vi "Routing Channel Page.vi"(8 "error in (no error)":errorcluster, 11 "Node Ptr":T6 format="%.0x") -> (0 "error out":errorcluster)   [LabVIEW 2020, in "Routing and Faulting System Explorer.lvlib"]
uses:
  Routing and Faulting System Explorer.lvlib
  <vilib>/NI VeriStand/Custom Device API/Custom Device API.lvlib
  Scripting/Routing and Faulting Scripting.lvlib
  Routing Channel Page Controls.ctl
  Shared/UI Common/UI Common.lvlib
  2402a215-ce2b-4427-ab28-3f6d8102afb6.vi
  Shared/Constants.vi
  Shared/Routing and Faulting Shared.lvlib
  <vilib>/NI VeriStand/Custom Device API/Custom Device Item Ref.ctl
  State Control.ctl
  State-Value Row.ctl
  Connection Row.ctl
  Shared/UI Common/Add Button.ctl
panel:
  in  "Configuration Tab":T1(tab)
  in  "Connections":T2[](array[typedef])
  in  "State Value":string
  in  "State Description":string
  in  "Add Connection":T3
  in  "State Name":T4
  in  "Duplicate State":bool
  in  "Remove State":bool
  in  "Add State":bool
  in  "Previous State":bool
  in  "Next State":bool
  in  "States":T5[](array[typedef])
  in  "Initial State":string(combo)
  in  "Routing Channel Name":string
  in  "SHDocVw.IWebBrowser":refnum<k7>(container)
  in  "Description":string
  # "Source"
  # "Destination"
  # "State Name"
  # "State Value"
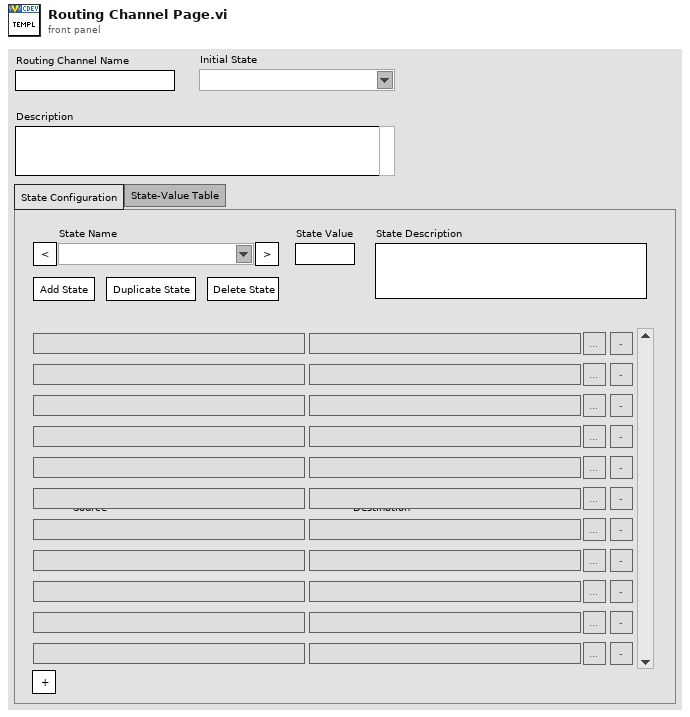
[diagram p1: front panel]
types:
  T1 = enum32{"State Configuration", "State-Value Table"}
  T2 = typedef "Routing and Faulting System Explorer.lvlib/Connection Row.ctl" = cluster{"Source":string, "Destination":string, "Edit":bool, "Remove":bool}
  T3 = typedef "UI Common.lvlib/Add Button.ctl" = bool
  T4 = typedef "Routing and Faulting System Explorer.lvlib/State Control.ctl" = string
  T5 = typedef "Routing and Faulting System Explorer.lvlib/State-Value Row.ctl" = cluster{"State":string, "State Value":string}
  T6 = typedef "Custom Device API.lvlib/Custom Device Item Ref.ctl" = u64
  T7 = typedef "Routing and Faulting System Explorer.lvlib/Routing Channel Page Controls.ctl" = cluster{"Description":refnum<vi>, "Routing Channel Name":refnum<vi>, "Initial State":refnum<vi>, "Configuration Tab":refnum<vi>, "States":refnum<vi>, "State Value":refnum<vi>, "State Name":refnum<vi>, "State Description":refnum<vi>, "Connections":refnum<vi>}
  T8 = typedef "Routing and Faulting Scripting.lvlib/Module Information.ctl" = cluster{"Module Path":string, "Product Name":string, "Possible Connections":T9[], "Configuration Revision":u32, "Validated":bool, "Missing":bool}
  T9 = typedef "Routing and Faulting Hardware API.lvlib/Possible Connections for Endpoint.ctl" = cluster{"Source":string, "Destinations":string[]}
  T10 = typedef "Routing and Faulting System Explorer.lvlib/Channel Editor State.ctl" = cluster{"Modules and Connections":T11[], "Alias Mappings UI":T12[], "Mappings by Module UI":T14[]}
  T11 = typedef "Routing and Faulting System Explorer.lvlib/Possible Connections.ctl" = cluster{" Module Path":string, "Short Module Path":string, "Product Name":string, "Possible Connections":T9[], "Missing":bool}
  T12 = typedef "Routing and Faulting Shared.lvlib/Alias Mapping.ctl" = cluster{"Alias":string, "Endpoint":T13}
  T13 = typedef "Routing and Faulting Shared.lvlib/Alias Endpoint.ctl" = cluster{"Module Path":string, "Endpoint":string}
  T14 = typedef "Routing and Faulting System Explorer.lvlib/Alias Map by Module.ctl" = cluster{"Module":string, "Alias Map":cluster{"Aliases":string[], "Endpoints":string[]}}
  T15 = typedef "Custom Device API.lvlib/Custom Device Commands.ctl" = enum16{"Default", "Item renamed", "Shutdown", "Dynamic button pressed"}
  T16 = typedef "Routing and Faulting Shared.lvlib/Connection.ctl" = cluster{"Module":string, "Source":string, "Destination":string}
  T17 = typedef "LVPoint32TypeDef.ctl" = cluster{"Horizontal":i32, "Vertical":i32}
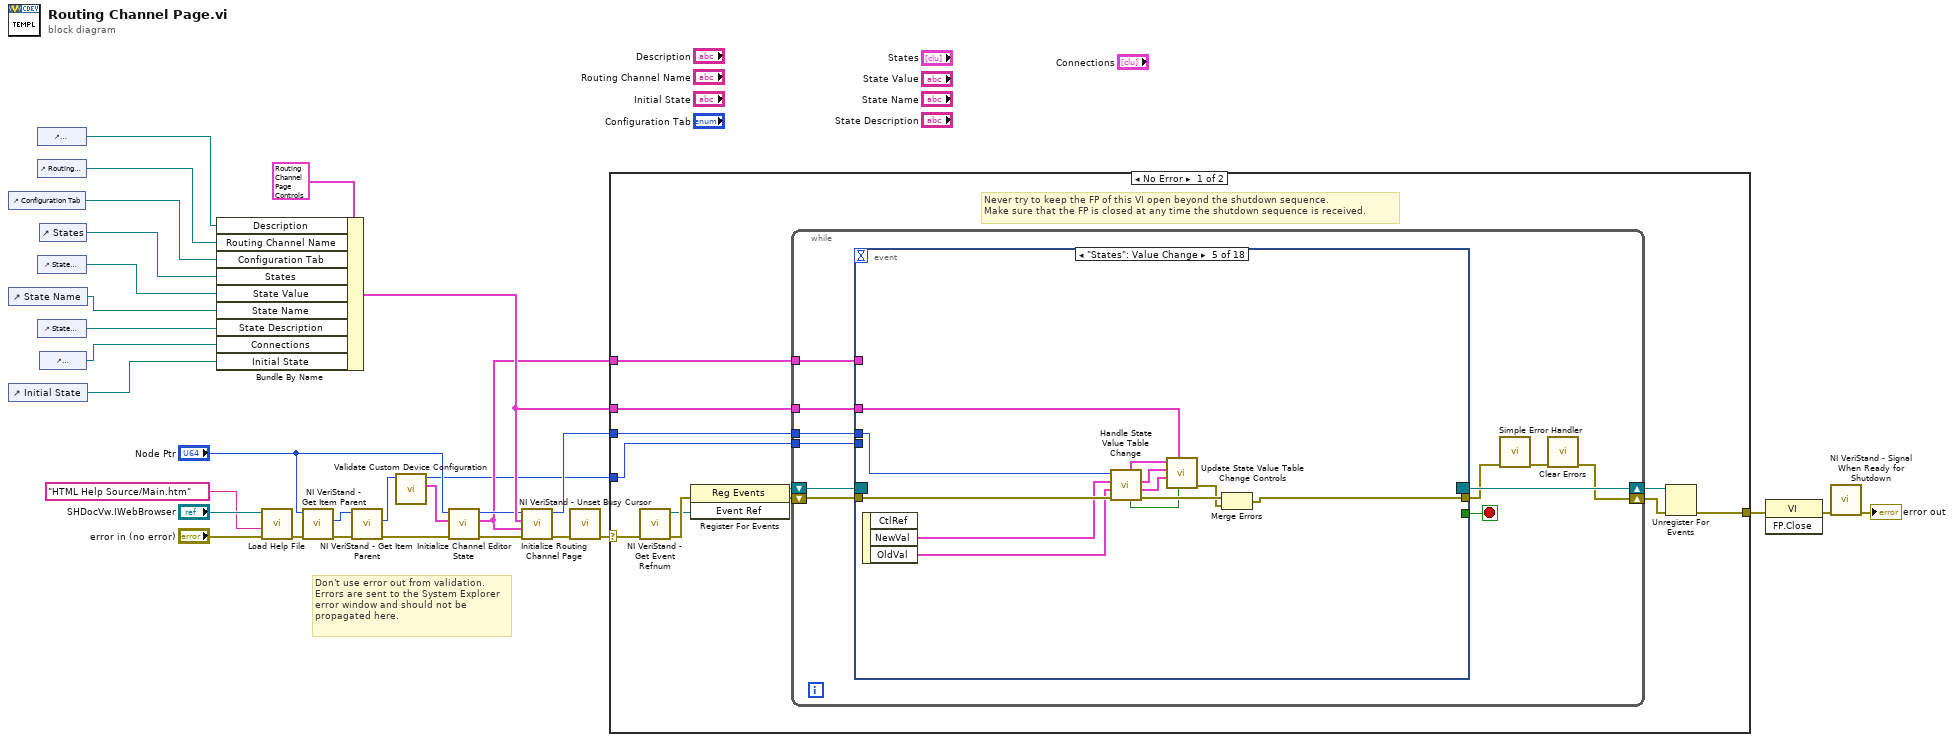
[diagram p0: block diagram]
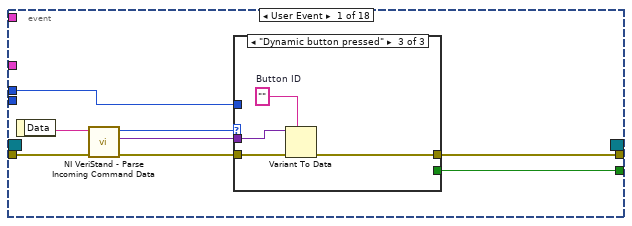
[diagram p2: hidden frame]
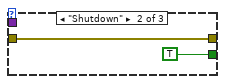
[diagram p4: hidden frame]
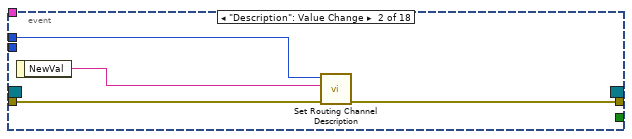
[diagram p5: hidden frame]
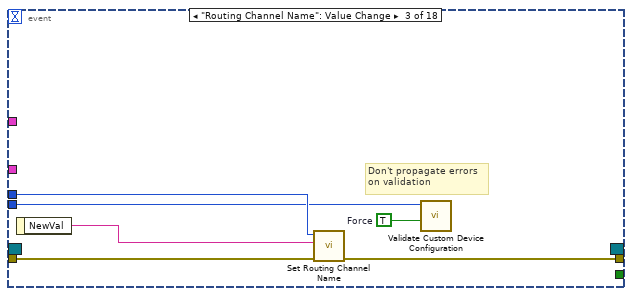
[diagram p6: hidden frame]
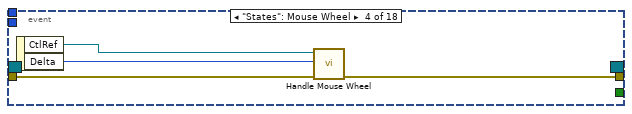
[diagram p7: hidden frame]
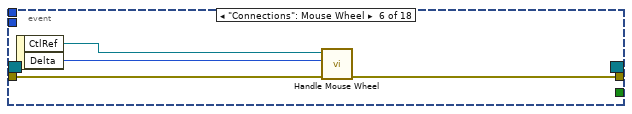
[diagram p8: hidden frame]
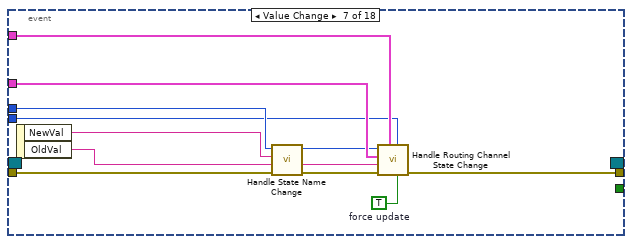
[diagram p9: hidden frame]
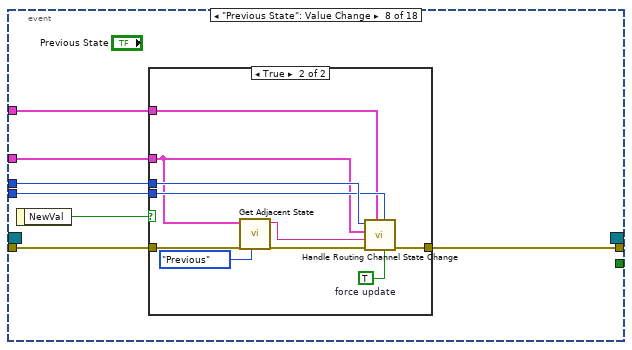
[diagram p10: hidden frame]
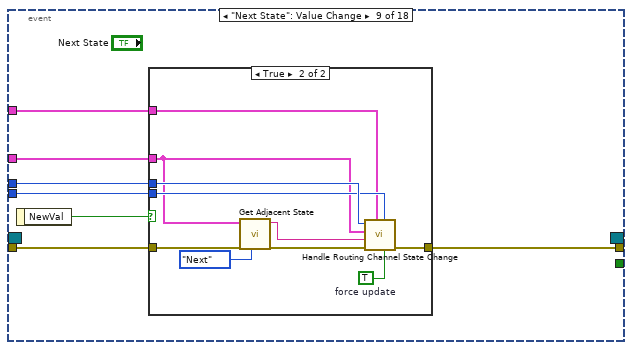
[diagram p12: hidden frame]
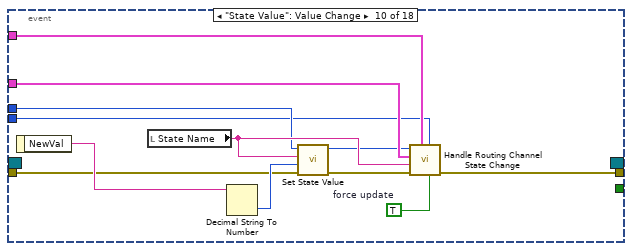
[diagram p14: hidden frame]
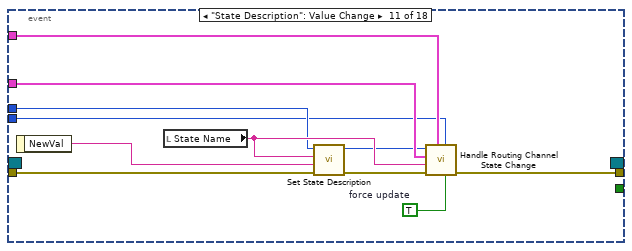
[diagram p15: hidden frame]
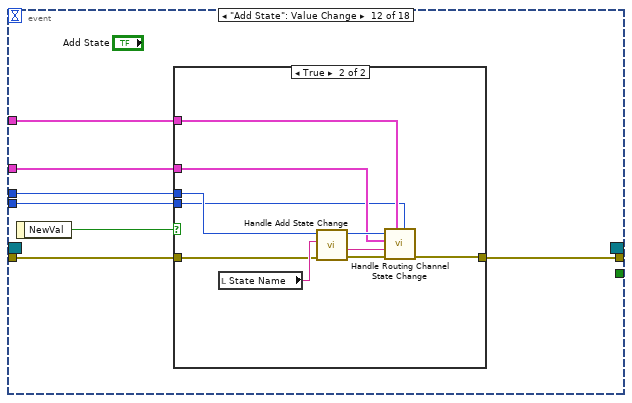
[diagram p16: hidden frame]
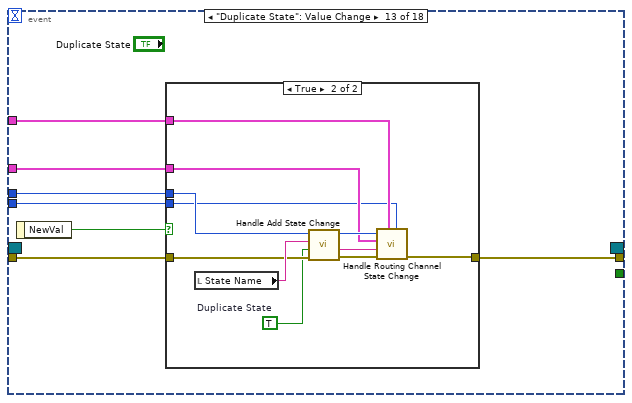
[diagram p18: hidden frame]
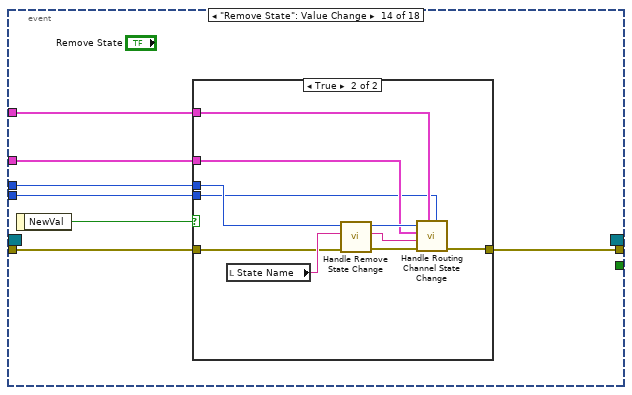
[diagram p20: hidden frame]
diagram:
  # "Don't use error out from validation.\nErrors are sent to the System Explorer\nerror window and should not be\npropagated here."
  n1 = control-ref of="Configuration Tab"() -> (w26:refnum<vi>)
  n2 = control-ref of="State Name"() -> (w18:refnum<vi>)
  n3 = control-ref of="Initial State"() -> (w14:refnum<vi>)
  n4 = control-ref of="Description"() -> (w27:refnum<vi>)
  n5 = control-ref of="Routing Channel Name"() -> (w12:refnum<vi>)
  n6 = control-ref of="State Value"() -> (w24:refnum<vi>)
  n7 = control-ref of="State Description"() -> (w13:refnum<vi>)
  n8 = control-ref of="States"() -> (w25:refnum<vi>)
  n9 = control-ref of="Connections"() -> (w19:refnum<vi>)
  n10 = Bundle By Name(cluster=T7 {"Description"=refnum, "Routing Channel Name"=refnum, "Initial State"=refnum, "Configuration Tab"=refnum, "States"=refnum, "State Value"=refnum, "State Name"=refnum, "State Description"=refnum, "Connections"=refnum} ("Routing Channel Page Controls"), "Description"=w27, "Routing Channel Name"=w12, "Configuration Tab"=w26, "States"=w25, "State Value"=w24, "State Name"=w18, "State Description"=w13, "Connections"=w19, "Initial State"=w14) -> (w15:T7)
  n11 = call "Load Help File.vi"("error in (no error)"="error in (no error)", "HTML File to Load"="HTML Help Source/Main.htm" ("HTML File"), "Browser"="SHDocVw.IWebBrowser") -> ("error out"=w6:errorcluster)  [unwired: 8 in]
  n12 = call <vilib>:"NI VeriStand - Get Item Parent.vi"("error in (no error)"=w6, "Item Ref in"="Node Ptr") -> ("error out"=w7:errorcluster, "Parent Ref"=w8:T6)  [unwired: 6 in, 2 out]
  n13 = call <vilib>:"NI VeriStand - Get Item Parent.vi"("error in (no error)"=w7, "Item Ref in"=w8) -> ("error out"=w5:errorcluster, "Parent Ref"=w3:T6)  [unwired: 6 in, 2 out]
  n14 = call "Validate Custom Device Configuration.vi"("Routing and Faulting Custom Device Ref"=w3) -> ("Module Connection Information"=w4:T8[], "Routing and Faulting Custom Device Ref out"=w1:T6)  [unwired: 8 in, 1 out]
  n15 = call "Initialize Channel Editor State.vi"("error in (no error)"=w5, "Module Connection Information"=w4, "Routing Channel Ref in"="Node Ptr") -> ("error out"=w10:errorcluster, "Channel Editor State"=w9:T10, "Routing Channel Ref out"=w11:T6)  [unwired: 6 in]
  n16 = call "Initialize Routing Channel Page.vi"("error in (no error)"=w10, "Channel Editor State"=w9, "Routing Channel Page Controls"=w15, "Routing Channel Ref in"=w11) -> ("error out"=w16:errorcluster, "Routing Channel Ref out"=w17:T6)  [unwired: 6 in]
  n17 = call <vilib>:"NI VeriStand - Unset Busy Cursor.vi"("error in (no error)"=w16) -> ("error out"=w28:errorcluster)  [unwired: 10 out]
  n18 = case shown="No Error" w28 {
    selector: w28 -> [w35 w298]
    tunnel: [w40 w296] -> w31
    tunnel: w17 -> [w36 _]
    tunnel: w15 -> [w34 _]
    tunnel: w9 -> [w33 _]
    tunnel: w1 -> [w32 _]
    frame No Error {
      # "Never try to keep the FP of this VI open beyond the shutdown sequence.\nMake sure that the FP is closed at any time the shutdown sequence is received."
      n19 = call <vilib>:"NI VeriStand - Get Event Refnum.vi"("error in (no error)"=w35) -> ("error out"=w43:errorcluster, "Event Ref"=w39:refnum<user-event>)  [unwired: 9 out]
      n20 = register-events(error in=w43, w39) -> (reference out=w37:refnum<event-registration>, error out=w38:errorcluster)  [unwired: 1 in]
      n21 = while {
        tunnel: w36 -> [w50]
        shift-right: [w47] -> w41
        shift-left: w38 -> [w53]
        shift-right: [w54] -> w42
        shift-left: w37 -> [w52]
        tunnel: w34 -> [w46]
        tunnel: w33 -> [w45]
        tunnel: w32 -> [w44]
        stop <- w51 stop-if-true
        n22 = event shown="[4] \"States\": Value Change" {
          selector: w52 -> [_ _ _ _ _ _ _ _ _ _ _ _ _ _ _ _ _ _]
          dyn-events: [_ _ _ _ _ _ _ _ _ _ _ _ _ _ _ _ _ _] -> w54
          timeout: _ -> [_ _ _ _ _ _ _ _ _ _ _ _ _ _ _ _ _ _]
          tunnel: w53 -> [w62 w72 w78 w82 w95 w98 w109 w118 w136 w155 w168 w176 w194 w212 w234 w242 _ w295]
          tunnel: [w58 _ _ _ _ _ _ _ _ _ _ _ _ _ _ _ _ _] -> w51
          tunnel: [w57 w71 w74 w83 w85 w99 w111 w117 w135 w159 w170 w175 w193 w211 w233 w240 _ w288] -> w49
          tunnel: w50 -> [w56 w73 w79 _ w91 _ w106 w114 w132 w152 w165 w177 w195 w214 w230 w244 _ w293]
          tunnel: w46 -> [_ _ _ _ w89 _ w110 w115 w133 w158 w169 w173 w191 w213 w235 w241 _ w286]
          tunnel: w45 -> [_ _ _ _ _ _ w101 w113 w131 w149 w161 w172 w190 w209 w227 w237 w259 w282]
          tunnel: w44 -> [_ _ w76 _ _ _ w100 w112 w130 w148 w160 w171 w189 w208 w226 w236 _ w281]
          event User Event {
            n23 = event-data() -> ("Data"=w61:string)  [unwired: 1 out]
            n24 = call <vilib>:"NI VeriStand - Parse Incoming Command Data.vi"("error in (no error)"=w62, "Incoming data"=w61) -> ("error out"=w60:errorcluster, "Outgoing data"=w55:variant, "Action"=w59:T15)  [unwired: 7 out]
            n25 = case shown="\"Dynamic button pressed\"" w59 {
              tunnel: w60 -> [w63 w64 w69]
              tunnel: [_ TRUE _] -> w58
              tunnel: [w63 w64 w66] -> w57
              tunnel: w56 -> [_ _ _]
              tunnel: w55 -> [_ _ w68]
              frame "Default", Default {
              }
              frame "Shutdown" {
              }
              frame "Dynamic button pressed" {
                w67 = ""  # Button ID
                n26 = Variant To Data(error in=w69, type=w67, Variant=w68) -> (error out=w66:errorcluster)  [unwired: 1 out]
              }
            }
          }
          event "Description": Value Change {
            n27 = event-data() -> ("NewVal"=w70:string)  [unwired: 1 out]
            n28 = call "Set Routing Channel Description.vi"("error in"=w72, "description"=w70, "routing channel in"=w73) -> ("error out"=w71:errorcluster)  [unwired: 7 in, 1 out]
          }
          event "Routing Channel Name": Value Change {
            w75 = TRUE  # Force
            # "Don't propagate errors\non validation"
            n29 = event-data() -> ("NewVal"=w77:string)  [unwired: 1 out]
            n30 = call "Set Routing Channel Name.vi"("error in"=w78, "routing channel name"=w77, "routing channel in"=w79) -> ("error out"=w74:errorcluster)  [unwired: 7 in, 1 out]
            n31 = call "Validate Custom Device Configuration.vi"("Force Validation (F)"=w75, "Routing and Faulting Custom Device Ref"=w76) -> ()  [unwired: 7 in, 3 out]
          }
          event "States": Mouse Wheel {
            n32 = event-data() -> ("CtlRef"=w81:refnum<vi>, "Delta"=w80:i32)  [unwired: 1 out]
            n33 = call "Handle Mouse Wheel.vi"("error in (no error)"=w82, "delta"=w80, "Array Refnum"=w81) -> ("error out"=w83:errorcluster)  [unwired: 7 in, 1 out]
          }
          event "States": Value Change {
            n34 = event-data() -> ("NewVal"=w93:T5[], "OldVal"=w92:T5[])  [unwired: 2 out]
            n35 = call "Handle State Value Table Change.vi"("error in (no error)"=w95, "OldVal"=w92, "NewVal"=w93, "routing channel in"=w91) -> ("error out"=w94:errorcluster, "old modified state and value"=w87:T5, "new modified state and value"=w88:T5, "update controls"=w86:bool, "coerced newval"=w90:T5[])  [unwired: 2 in, 1 out]
            n36 = call "Update State Value Table Change Controls.vi"("update all controls?"=w86, "Routing Channel Page Controls"=w89, "old modified state and value"=w87, "new modified state and value"=w88, "all states and values"=w90) -> ("error out"=w84:errorcluster)  [unwired: 6 in]
            n37 = Merge Errors(w94, w84) -> (w85:errorcluster)
          }
          event "Connections": Mouse Wheel {
            n38 = event-data() -> ("CtlRef"=w96:refnum<vi>, "Delta"=w97:i32)  [unwired: 1 out]
            n39 = call "Handle Mouse Wheel.vi"("error in (no error)"=w98, "delta"=w97, "Array Refnum"=w96) -> ("error out"=w99:errorcluster)  [unwired: 7 in, 1 out]
          }
          event Value Change {
            w102 = TRUE  # force update
            n40 = event-data() -> ("NewVal"=w108:T4, "OldVal"=w107:T4)  [unwired: 1 out]
            n41 = call "Handle State Name Change.vi"("error in (no error)"=w109, "Old State Name"=w107, "New State Name"=w108, "Routing Channel Ref in"=w106) -> ("error out"=w105:errorcluster, "State to Display"=w103:string, "Routing Channel Ref out"=w104:T6)  [unwired: 5 in]
            n42 = call "Handle Routing Channel State Change.vi"("force update"=w102, "Routing and Faulting Custom Device Ref"=w100, "Channel Editor State"=w101, "error in (no error)"=w105, "State"=w103, "Routing Channel Page Controls"=w110, "Routing Channel Ref in"=w104) -> ("error out"=w111:errorcluster)  [unwired: 3 in, 1 out]
          }
          event "Previous State": Value Change {
            n43 = event-data() -> ("NewVal"=w116:bool)  [unwired: 1 out]
            n44 = case shown="True" w116 {
              tunnel: w118 -> [w119 w122]
              tunnel: [w119 w128] -> w117
              tunnel: w115 -> [_ w124]
              tunnel: w114 -> [_ w127]
              tunnel: w113 -> [_ w125]
              tunnel: w112 -> [_ w126]
              frame False {
              }
              frame True {
                w129 = TRUE  # force update
                n45 = call "Get Adjacent State.vi"("Direction"=enum16{"Previous", "Next"}."Previous", "error in (no error)"=w122, "Routing Channel Page Controls"=w124) -> ("error out"=w123:errorcluster, "state name"=w121:string)  [unwired: 7 in]
                n46 = call "Handle Routing Channel State Change.vi"("force update"=w129, "Routing and Faulting Custom Device Ref"=w126, "Channel Editor State"=w125, "error in (no error)"=w123, "State"=w121, "Routing Channel Page Controls"=w124, "Routing Channel Ref in"=w127) -> ("error out"=w128:errorcluster)  [unwired: 3 in, 1 out]
              }
            }
          }
          event "Next State": Value Change {
            n47 = event-data() -> ("NewVal"=w134:bool)  [unwired: 1 out]
            n48 = case shown="True" w134 {
              tunnel: w136 -> [w137 w140]
              tunnel: [w137 w146] -> w135
              tunnel: w133 -> [_ w142]
              tunnel: w132 -> [_ w145]
              tunnel: w131 -> [_ w143]
              tunnel: w130 -> [_ w144]
              frame False {
              }
              frame True {
                w147 = TRUE  # force update
                n49 = call "Get Adjacent State.vi"("Direction"=enum16{"Previous", "Next"}."Next", "error in (no error)"=w140, "Routing Channel Page Controls"=w142) -> ("error out"=w141:errorcluster, "state name"=w139:string)  [unwired: 7 in]
                n50 = call "Handle Routing Channel State Change.vi"("force update"=w147, "Routing and Faulting Custom Device Ref"=w144, "Channel Editor State"=w143, "error in (no error)"=w141, "State"=w139, "Routing Channel Page Controls"=w142, "Routing Channel Ref in"=w145) -> ("error out"=w146:errorcluster)  [unwired: 3 in, 1 out]
              }
            }
          }
          event "State Value": Value Change {
            w150 = TRUE  # force update
            n51 = event-data() -> ("NewVal"=w156:string)  [unwired: 1 out]
            n52 = local read "State Name"() -> (w153:T4)
            n53 = Decimal String To Number(string=w156) -> (number=w157:i32)  [unwired: 2 in, 1 out]
            n54 = call "Set State Value.vi"("error in"=w155, "value"=w157, "state"=w153, "routing channel in"=w152) -> ("error out"=w154:errorcluster, "routing channel out"=w151:T6)  [unwired: 6 in]
            n55 = call "Handle Routing Channel State Change.vi"("force update"=w150, "Routing and Faulting Custom Device Ref"=w148, "Channel Editor State"=w149, "error in (no error)"=w154, "State"=w153, "Routing Channel Page Controls"=w158, "Routing Channel Ref in"=w151) -> ("error out"=w159:errorcluster)  [unwired: 3 in, 1 out]
          }
          event "State Description": Value Change {
            w163 = TRUE  # force update
            n56 = event-data() -> ("NewVal"=w162:string)  [unwired: 1 out]
            n57 = local read "State Name"() -> (w166:T4)
            n58 = call "Set State Description.vi"("error in"=w168, "descriptions"=w162, "state"=w166, "routing channel in"=w165) -> ("error out"=w167:errorcluster, "routing channel out"=w164:T6)  [unwired: 6 in]
            n59 = call "Handle Routing Channel State Change.vi"("force update"=w163, "Routing and Faulting Custom Device Ref"=w160, "Channel Editor State"=w161, "error in (no error)"=w167, "State"=w166, "Routing Channel Page Controls"=w169, "Routing Channel Ref in"=w164) -> ("error out"=w170:errorcluster)  [unwired: 3 in, 1 out]
          }
          event "Add State": Value Change {
            n60 = event-data() -> ("NewVal"=w174:bool)  [unwired: 1 out]
            n61 = case shown="True" w174 {
              tunnel: w177 -> [_ w188]
              tunnel: w173 -> [_ w184]
              tunnel: w176 -> [w178 w182]
              tunnel: [w178 w183] -> w175
              tunnel: w172 -> [_ w180]
              tunnel: w171 -> [_ w179]
              frame False {
              }
              frame True {
                n62 = local read "State Name"() -> (w187:T4)
                n63 = call "Handle Add State Change.vi"("error in (no error)"=w182, "State"=w187, "Routing Channel Ref in"=w188) -> ("error out"=w185:errorcluster, "New State Added"=w181:string, "Routing Channel Ref out"=w186:T6)  [unwired: 6 in]
                n64 = call "Handle Routing Channel State Change.vi"("Routing and Faulting Custom Device Ref"=w179, "Channel Editor State"=w180, "error in (no error)"=w185, "State"=w181, "Routing Channel Page Controls"=w184, "Routing Channel Ref in"=w186) -> ("error out"=w183:errorcluster)  [unwired: 4 in, 1 out]
              }
            }
          }
          event "Duplicate State": Value Change {
            n65 = event-data() -> ("NewVal"=w192:bool)  [unwired: 1 out]
            n66 = case shown="True" w192 {
              tunnel: w195 -> [_ w207]
              tunnel: w191 -> [_ w203]
              tunnel: w194 -> [w196 w201]
              tunnel: [w196 w202] -> w193
              tunnel: w190 -> [_ w198]
              tunnel: w189 -> [_ w197]
              frame False {
              }
              frame True {
                w199 = TRUE  # Duplicate State
                n67 = local read "State Name"() -> (w206:T4)
                n68 = call "Handle Add State Change.vi"("error in (no error)"=w201, "Duplicate State"=w199, "State"=w206, "Routing Channel Ref in"=w207) -> ("error out"=w204:errorcluster, "New State Added"=w200:string, "Routing Channel Ref out"=w205:T6)  [unwired: 5 in]
                n69 = call "Handle Routing Channel State Change.vi"("Routing and Faulting Custom Device Ref"=w197, "Channel Editor State"=w198, "error in (no error)"=w204, "State"=w200, "Routing Channel Page Controls"=w203, "Routing Channel Ref in"=w205) -> ("error out"=w202:errorcluster)  [unwired: 4 in, 1 out]
              }
            }
          }
          event "Remove State": Value Change {
            n70 = event-data() -> ("NewVal"=w210:bool)  [unwired: 1 out]
            n71 = case shown="True" w210 {
              tunnel: w214 -> [_ w225]
              tunnel: w213 -> [_ w221]
              tunnel: w212 -> [w215 w219]
              tunnel: [w215 w220] -> w211
              tunnel: w209 -> [_ w217]
              tunnel: w208 -> [_ w216]
              frame False {
              }
              frame True {
                n72 = local read "State Name"() -> (w224:T4)
                n73 = call "Handle Remove State Change.vi"("error in (no error)"=w219, "State"=w224, "Routing Channel Ref in"=w225) -> ("error out"=w222:errorcluster, "State to Display"=w218:string, "Routing Channel Ref out"=w223:T6)  [unwired: 6 in]
                n74 = call "Handle Routing Channel State Change.vi"("Routing and Faulting Custom Device Ref"=w216, "Channel Editor State"=w217, "error in (no error)"=w222, "State"=w218, "Routing Channel Page Controls"=w221, "Routing Channel Ref in"=w223) -> ("error out"=w220:errorcluster)  [unwired: 4 in, 1 out]
              }
            }
          }
          event "Initial State": Value Change {
            n75 = event-data() -> ("NewVal"=w228:string)  [unwired: 1 out]
            n76 = call "Set Routing Channel Initial State.vi"("error in"=w234, "state"=w228, "routing channel in"=w230) -> ("error out"=w231:errorcluster, "routing channel out"=w229:T6)  [unwired: 7 in]
            n77 = local read "State Name"() -> (w232:T4)
            n78 = call "Handle Routing Channel State Change.vi"("Routing and Faulting Custom Device Ref"=w226, "Channel Editor State"=w227, "error in (no error)"=w231, "State"=w232, "Routing Channel Page Controls"=w235, "Routing Channel Ref in"=w229) -> ("error out"=w233:errorcluster)  [unwired: 4 in, 1 out]
          }
          event Value Change {
            n79 = event-data() -> ()  [unwired: 2 out]
            n80 = call "Configure Connection Dialog.vi"("error in (no error)"=w242, "Channel Editor State"=w237) -> ("error out"=w243:errorcluster, "Connection (R,S,D)"=w238:T16, "Canceled?"=w239:bool)  [unwired: 7 in]
            n81 = case shown="False" w239 {
              tunnel: w244 -> [w252 _]
              tunnel: w238 -> [w248 _]
              tunnel: w243 -> [w249 w256]
              tunnel: w241 -> [w254 _]
              tunnel: [w251 w256] -> w240
              tunnel: w237 -> [w246 _]
              tunnel: w236 -> [w245 _]
              frame False {
                w247 = FALSE  # init index
                n82 = local read "State Name"() -> (w250:T4)
                n83 = call "Add Connection to State.vi"("error in"=w249, "connection"=w248, "state"=w250, "routing channel in"=w252) -> ("error out"=w255:errorcluster, "routing channel out"=w253:T6)  [unwired: 6 in]
                n84 = call "Handle Routing Channel State Change.vi"("Routing and Faulting Custom Device Ref"=w245, "init index"=w247, "Channel Editor State"=w246, "error in (no error)"=w255, "State"=w250, "Routing Channel Page Controls"=w254, "Routing Channel Ref in"=w253) -> ("error out"=w251:errorcluster)  [unwired: 3 in, 1 out]
              }
              frame True {
              }
            }
          }
          event "Connections": Mouse Move {
            n85 = event-data() -> ("CtlRef"=w260:refnum<vi>, "Coords"=w261:T17)  [unwired: 1 out]
            n86 = global read "Constants.vi" "Tip-Strip Update Period"() -> (w258:dbl)
            n87 = call "Elapsed Time"("Time Target (s)"=w258) -> ("Time has Elapsed"=w257:bool)  [unwired: 11 in, 7 out]
            n88 = case shown="True" w257 {
              tunnel: w261 -> [_ w268]
              tunnel: w260 -> [_ w267]
              tunnel: w259 -> [_ w266]
              frame False {
                # "Handle Mouse Move only every 10ms"
              }
              frame True {
                n89 = call "Get Mouse Location (Connections).vi"("Event Coord"=w268, "Connections Reference"=w267) -> ("in data range"=w262:bool, "Element Reference"=w263:refnum<vi>, "Type"=w265:enum16{"Source", "Destination", "Neither"}, "Array Index"=w264:i32)  [unwired: 6 in]
                n90 = case shown="\"Source\", \"Destination\"" w265 {
                  selector: w265 -> [_ w272]
                  tunnel: w266 -> [_ w273]
                  tunnel: w264 -> [_ w274]
                  tunnel: w263 -> [_ w270]
                  tunnel: w262 -> [_ w269]
                  frame Default {
                  }
                  frame "Source", "Destination" {
                    n91 = case shown="True" w269 {
                      tunnel: w274 -> [_ w279]
                      tunnel: w273 -> [_ w277]
                      tunnel: w272 -> [_ w276]
                      tunnel: [_ w275] -> w271
                      frame False {
                      }
                      frame True {
                        n92 = local read "Connections"() -> (w280:T2[])
                        n93 = Index Array(array=w280, index=w279) -> (element=w278:T2)
                        n94 = call "Get Alias-Free Connection Endpoint.vi"("type"=w276, "Connection row"=w278, "Channel Editor State"=w277) -> ("Endpoint (Model) String"=w275:string)  [unwired: 8 in]
                      }
                    }
                    n95 = property class="Ctl"(reference=w270, "TipStrip"=w271) -> ()  [unwired: 1 in, 2 out]
                  }
                }
              }
            }
          }
          event "Connections": Value Change {
            w283 = TRUE  # force update
            w290 = FALSE  # init index
            n96 = event-data() -> ("CtlRef"=w285:refnum<vi>, "NewVal"=w292:T2[], "OldVal"=w291:T2[])  [unwired: 1 out]
            n97 = call "Try Remove Array Element.vim"("error in (no error)"=w295, "Array"=w292, "Ctl Refnum"=w285) -> ("error out"=w294:errorcluster)  [unwired: 6 in, 2 out]
            n98 = local read "State Name"() -> (w284:T4)
            n99 = call "Handle Connections Value Change.vi"("State"=w284, "Channel Editor State"=w282, "error in (no error)"=w294, "OldVal"=w291, "NewVal"=w292, "Routing Channel Ref in"=w293) -> ("error out"=w289:errorcluster, "Routing Channel Ref out"=w287:T6)  [unwired: 4 in]
            n100 = call "Handle Routing Channel State Change.vi"("force update"=w283, "Routing and Faulting Custom Device Ref"=w281, "init index"=w290, "Channel Editor State"=w282, "error in (no error)"=w289, "State"=w284, "Routing Channel Page Controls"=w286, "Routing Channel Ref in"=w287) -> ("error out"=w288:errorcluster)  [unwired: 2 in, 1 out]
          }
        }
        n101 = call <vilib>:"Simple Error Handler.vi"("error in (no error)"=w49) -> ("error out"=w48:errorcluster)  [unwired: 1 in, 7 out]
        n102 = call <vilib>:"Clear Errors.vi"("error in (no error)"=w48) -> ("error out"=w47:errorcluster)  [unwired: 1 in, 5 out]
      }
      n103 = Unregister For Events(event registration refnum=w42, error in=w41) -> (error out=w40:errorcluster)
    }
    frame Error {
      n104 = call <vilib>:"Simple Error Handler.vi"("error in (no error)"=w298) -> ("error out"=w297:errorcluster)  [unwired: 1 in, 7 out]
      n105 = call <vilib>:"Clear Errors.vi"("error in (no error)"=w297) -> ("error out"=w296:errorcluster)  [unwired: 1 in, 5 out]
    }
  }
  n106 = invoke class="VI" method="FP.Close"(error in=w31) -> (error out=w30:errorcluster)  [unwired: 2 in, 2 out]
  n107 = call <vilib>:"NI VeriStand - Signal When Ready for Shutdown.vi"("error in (no error)"=w30) -> ("error out"=→"error out":errorcluster)  [unwired: 10 out]
